vi "lab2.vi"() -> ()   [LabVIEW 2025]
uses:
  <vilib>/Utility/NIReport.llb/Report Type.ctl
  <vilib>/addons/_office/excel.llb/Excel Get Data ([str]).vi
  <vilib>/Utility/NIReport.llb/NI_report.lvclass
  <vilib>/Utility/NIReport.llb/NI_ReportGenerationCore.lvlib
  <vilib>/Utility/NIReport.llb/Excel/NI_Excel.lvclass
  <vilib>/addons/_office/NI_ReportGenerationToolkit.lvlib
  <vilib>/measure/NI_MABase.lvlib
panel:
  out "Waveform Graph 3":dynamicdata(graph)
  in  "sampling info":cluster{"Fs":dbl, "#s":dbl}={"Fs"=1000.0, "#s"=1000.0} {"Fs" format="%.2p"}
  out "Waveform Graph":waveform(dbl)(graph)
  out "Forma de onda":string
  out "Voltaje (Vp)":string
  out "Frecuencia (Hz)":string
  out "data":string[][](array[string])
  in  "template":path
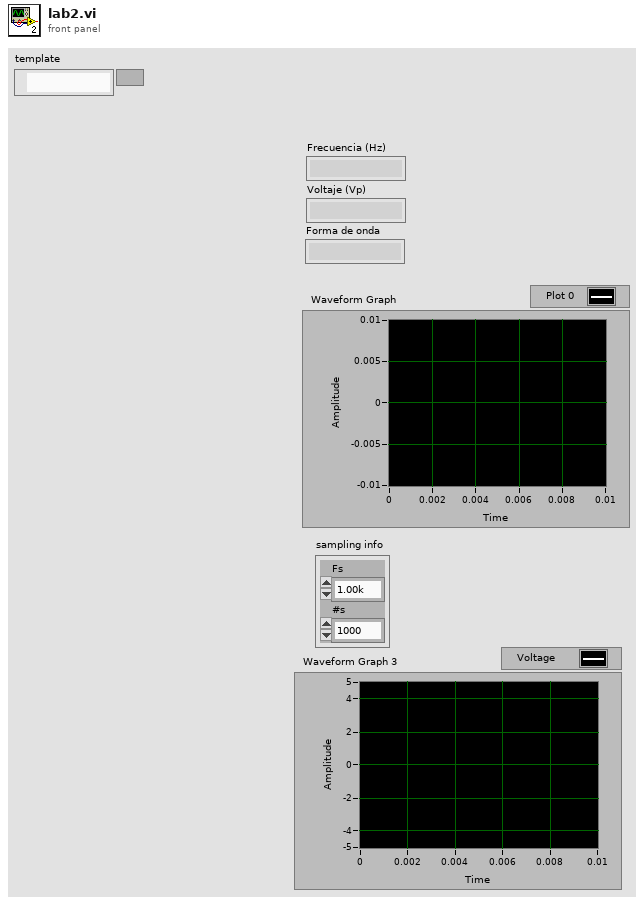
[diagram p1: front panel]
types:
  T1 = typedef "NI_ReportGenerationCore.lvlib/Report Type.ctl" = enum16{"HTML", "Word", "Excel"}
  T2 = enum16{"maximized", "minimized", "normal", "no change"}
  T3 = enum16{"Sine Wave", "Triangle Wave", "Square Wave", "Sawtooth Wave"}
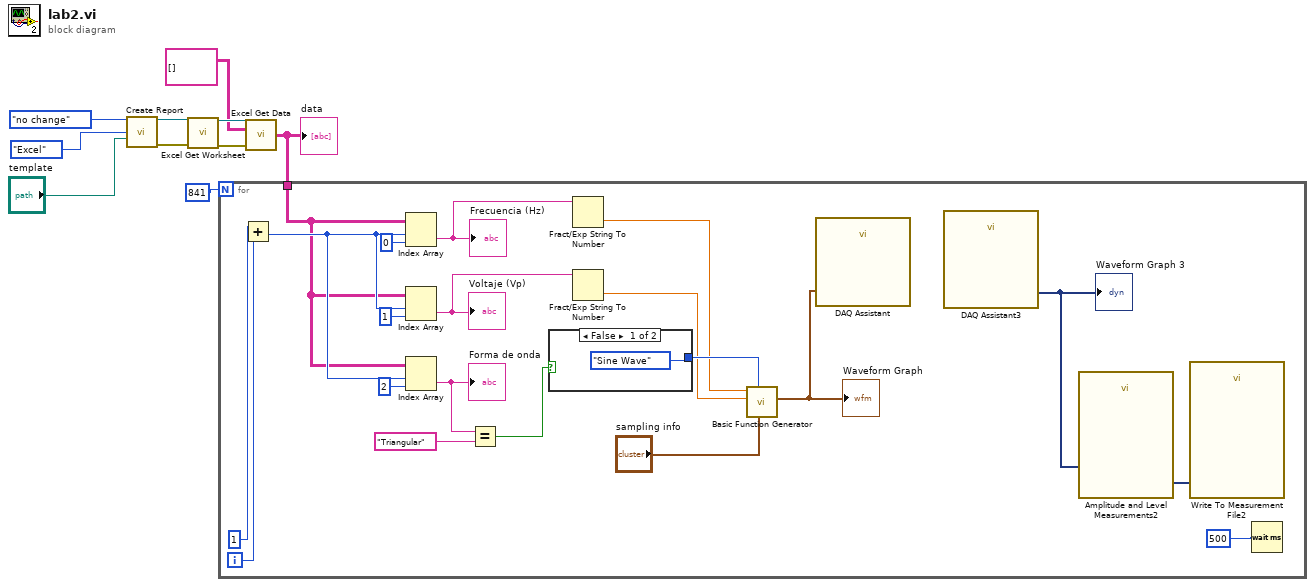
[diagram p0: block diagram]
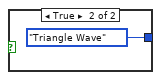
[diagram p2: hidden frame]
diagram:
  n1 = call <vilib>:"Create Report.vi"("window state (normal)"=T2."no change", "report type"=Report_Type."Excel", "template (empty)"="template") -> ("report out"=w7:refnum<class "NI_report.lvclass">, "error out"=w6:errorcluster)  [unwired: 11 in]
  n2 = call <vilib>:"Excel Get Worksheet.vi"("report in"=w7, "error in (no error)"=w6) -> ("report out"=w5:refnum<class "NI_report.lvclass">, "error out"=w4:errorcluster)  [unwired: 12 in]
  n3 = call-poly <vilib>:"Excel Get Data.vi"("report in"=w5, "data type"=string[][] [], "error in (no error)"=w4) -> ("data"=w1:string[][])  [unwired: 10 in, 2 out]
  "data" <- w1
  n4 = for {
    N: 841 -> [_]
    tunnel: w1 -> [w24]
    i -> [w29]
    n5 = Add(x=1, y=w29) -> (x+y=w26:i32)
    n6 = Index Array(array=w24, index (row)=w26, index (col)=0) -> (element=w23:string)
    "Frecuencia (Hz)" <- w23
    n7 = Index Array(array=w24, index (row)=w26, index (col)=1) -> (element=w22:string)
    "Voltaje (Vp)" <- w22
    n8 = Index Array(array=w24, index (row)=w26, index (col)=2) -> (element=w21:string)
    "Forma de onda" <- w21
    n9 = Equal?(x=w21, y="Triangular") -> (x = y?=w18:bool)
    n10 = case shown="False" w18 {
      tunnel: [T3."Sine Wave" ("signal type") T3."Triangle Wave" ("signal type")] -> w19
      frame False {
      }
      frame True {
      }
    }
    n11 = Fract/Exp String To Number(string=w23) -> (number=w17:dbl)  [unwired: 3 in, 1 out]
    n12 = Fract/Exp String To Number(string=w22) -> (number=w13:dbl)  [unwired: 3 in, 1 out]
    n13 = call <vilib>:"Basic Function Generator.vi"("sampling info"="sampling info", "signal type"=w19, "amplitude"=w13, "frequency"=w17) -> ("signal out"=w15:waveform(dbl))  [unwired: 5 in, 2 out]
    "Waveform Graph" <- w15
    n14 = call "DAQ Assistant"("data"=w15) -> ()  [unwired: 17 in, 2 out]
    n15 = call "DAQ Assistant3"() -> ("data"=w11:dynamicdata)  [unwired: 17 in, 2 out]
    "Waveform Graph 3" <- w11
    n16 = call "Amplitude and Level Measurements2"("Signals"=w11) -> ("Peak to Peak"=w12:dynamicdata)  [unwired: 13 in, 1 out]
    n17 = call "Write To Measurement File2"("Signals"=w12) -> ()  [unwired: 16 in, 3 out]
    n18 = Wait (ms)(milliseconds to wait=u32 500) -> ()  [unwired: 1 out]
  }
